vi "Curriculum Launcher.vi"(5 "Array of VISA Resources":refnum<visa-resource-name>[](array[refnum]), 7 "Device type":string[](array[string]), 8 "error in (no error)":errorcluster, 10 "Is the required hardware detected?":bool[](array[boolean]), 11 "Example File Paths":path[](array[path])) -> (0 "error out":errorcluster)   [LabVIEW 2020]
uses:
  <vilib>/Utility/sysdir.llb/System Directory Type.ctl
panel:
  in  "View Solution":bool
  in  "Multicolumn Listbox":i32(listbox)
  in  "Open Excercise Manual":bool
  in  "Open Button":bool
  # "If hardware is detected, the device references will be \npassed to the example."
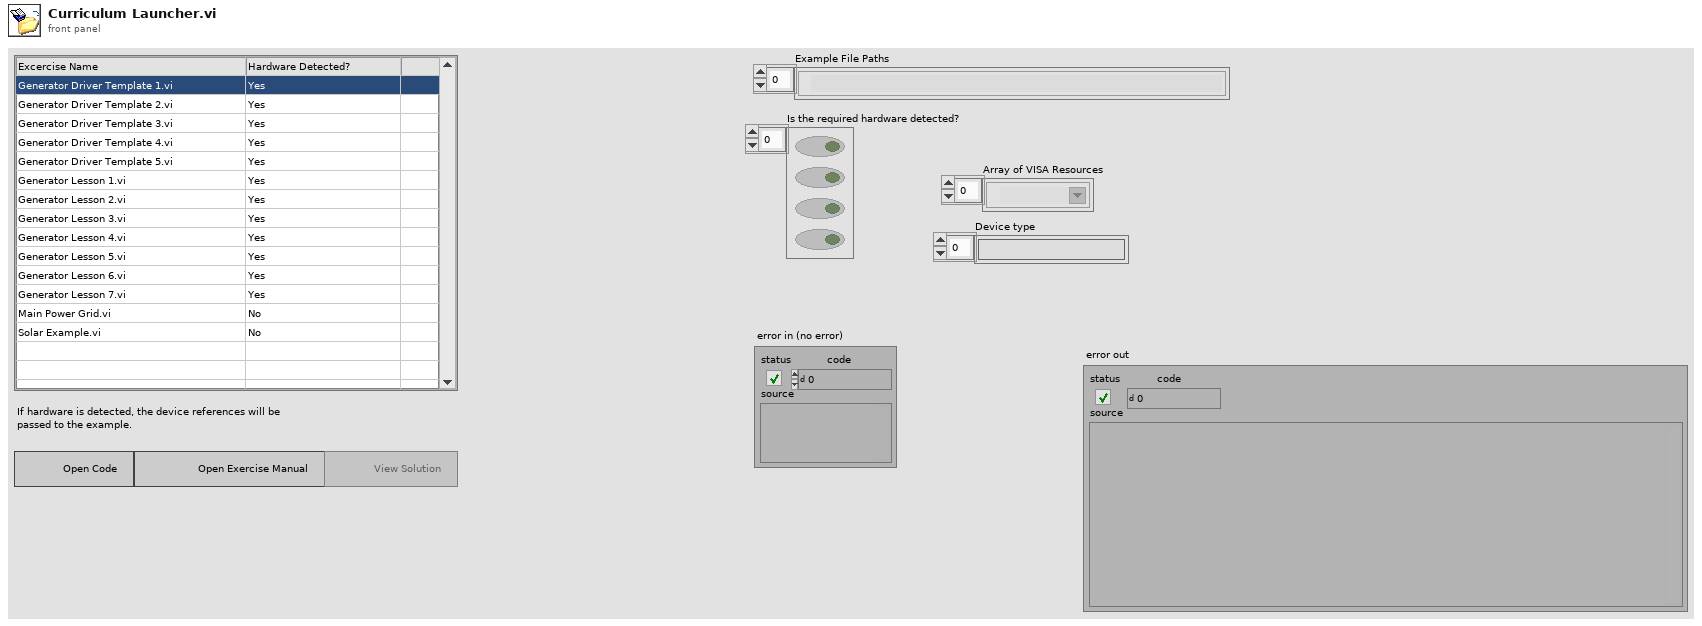
[diagram p1: front panel]
types:
  T1 = enum8{"Enabled", "Disabled", "Disabled and Grayed Out"}
  T2 = cluster{"Open Button":refnum<vi>, "Open Excercise Manual":refnum<vi>}
  T3 = enum32{"Invalid", "Standard", "Closed", "Hidden", "Minimized", "Maximized"}
  T4 = typedef "System Directory Type.ctl" = i32
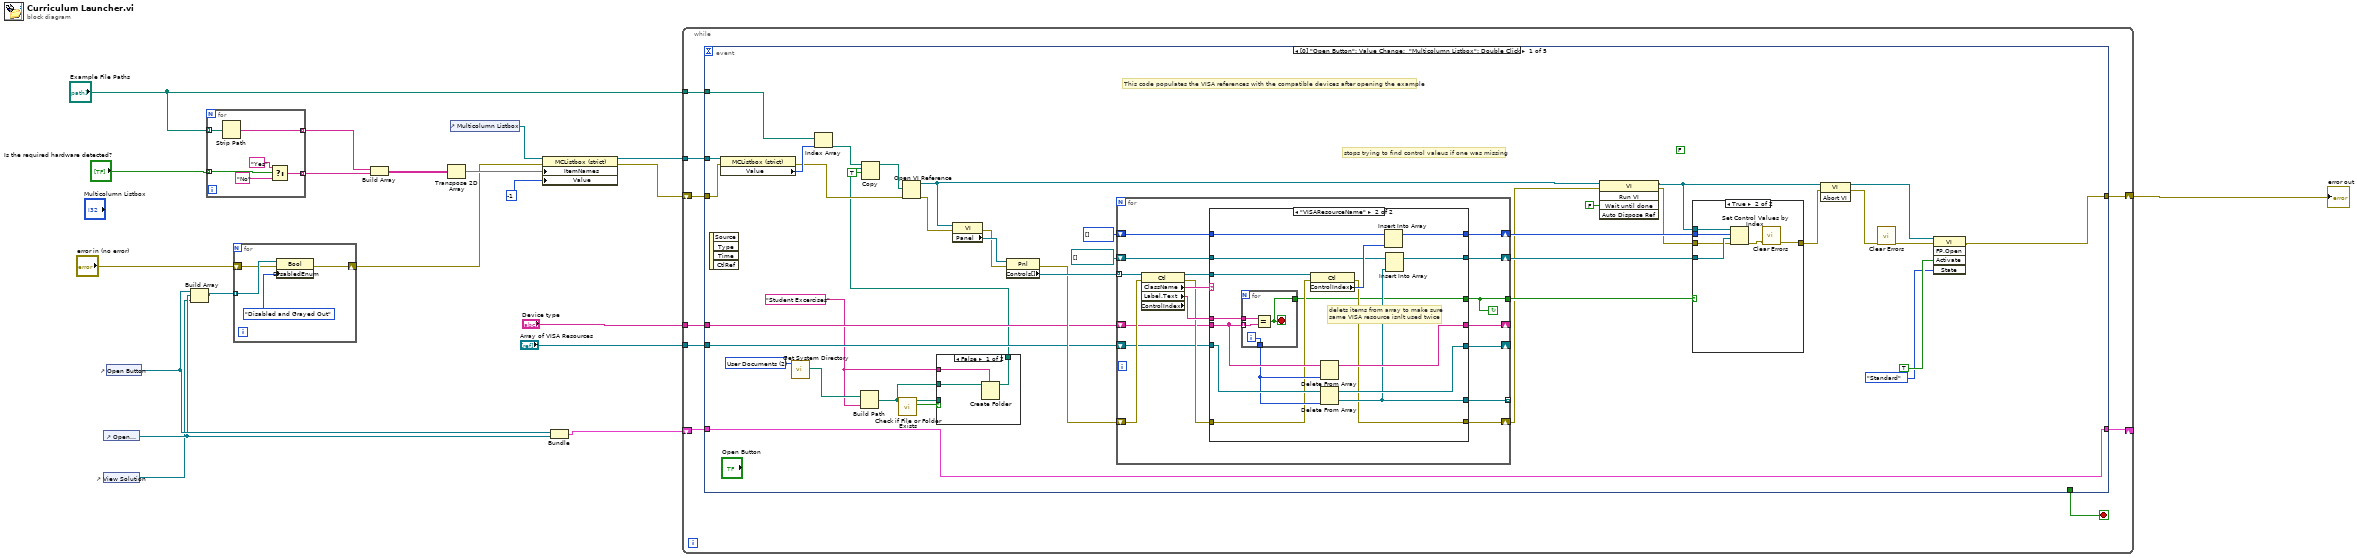
[diagram p0: block diagram]
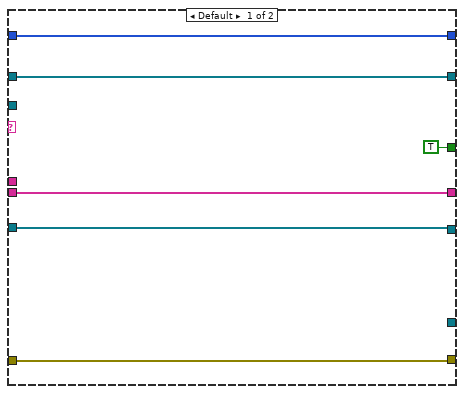
[diagram p4: hidden frame]
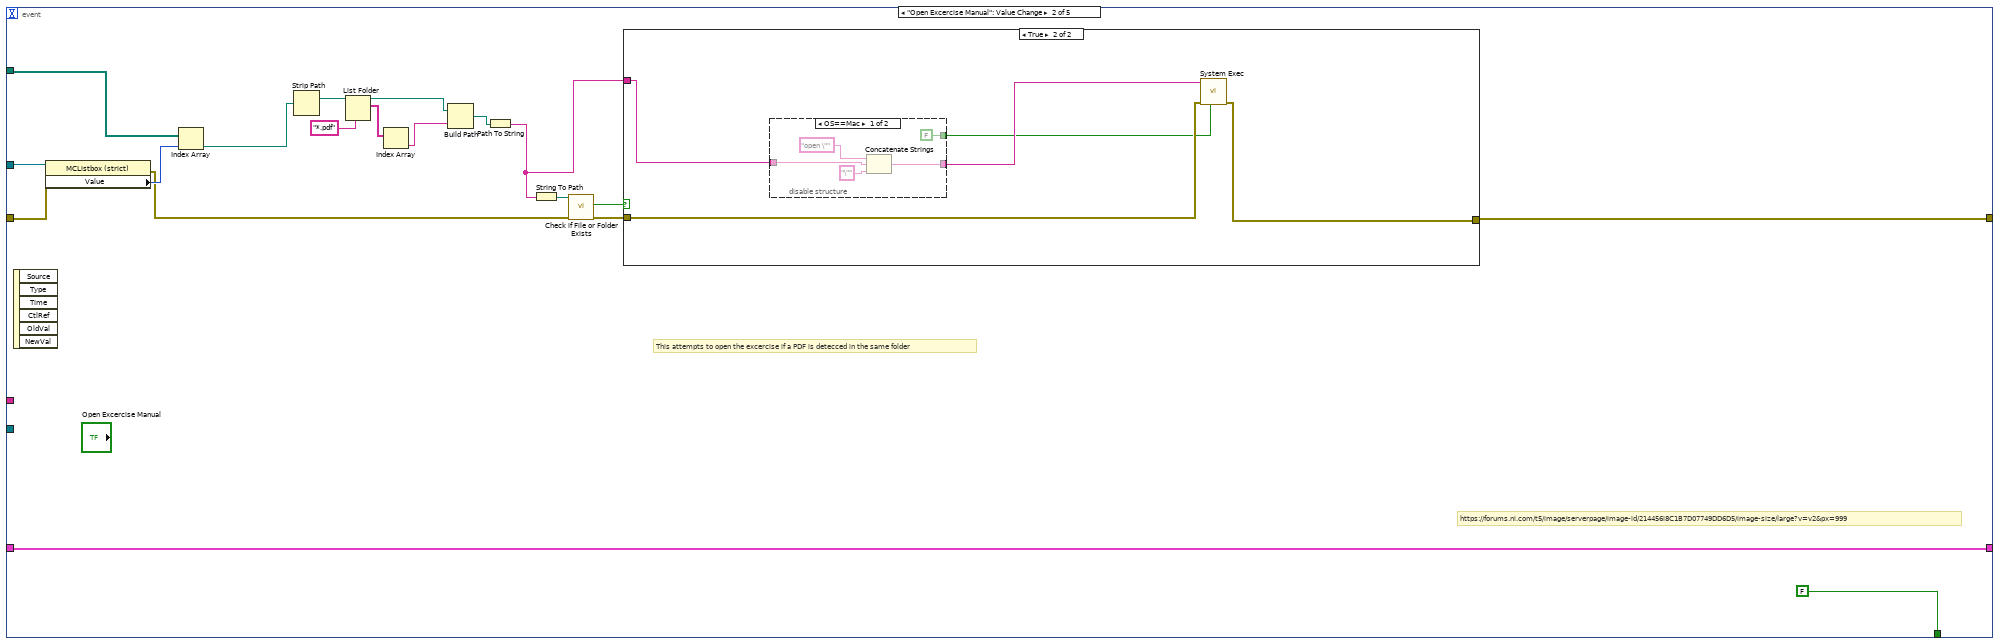
[diagram p5: hidden frame]
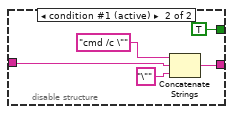
[diagram p7: hidden frame]
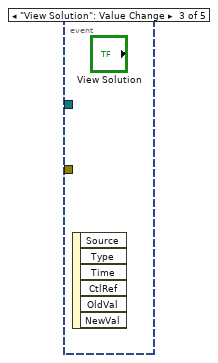
[diagram p8: hidden frame]
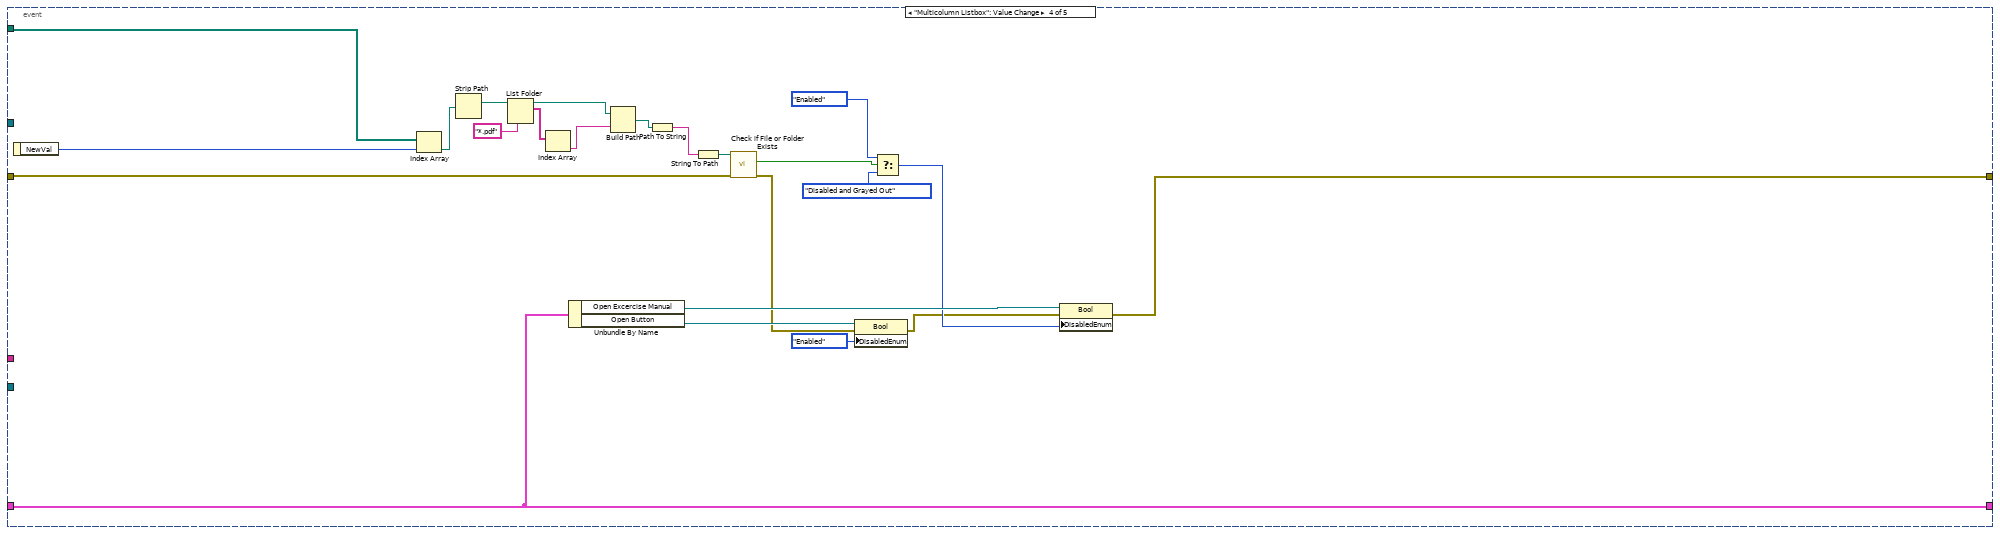
[diagram p9: hidden frame]
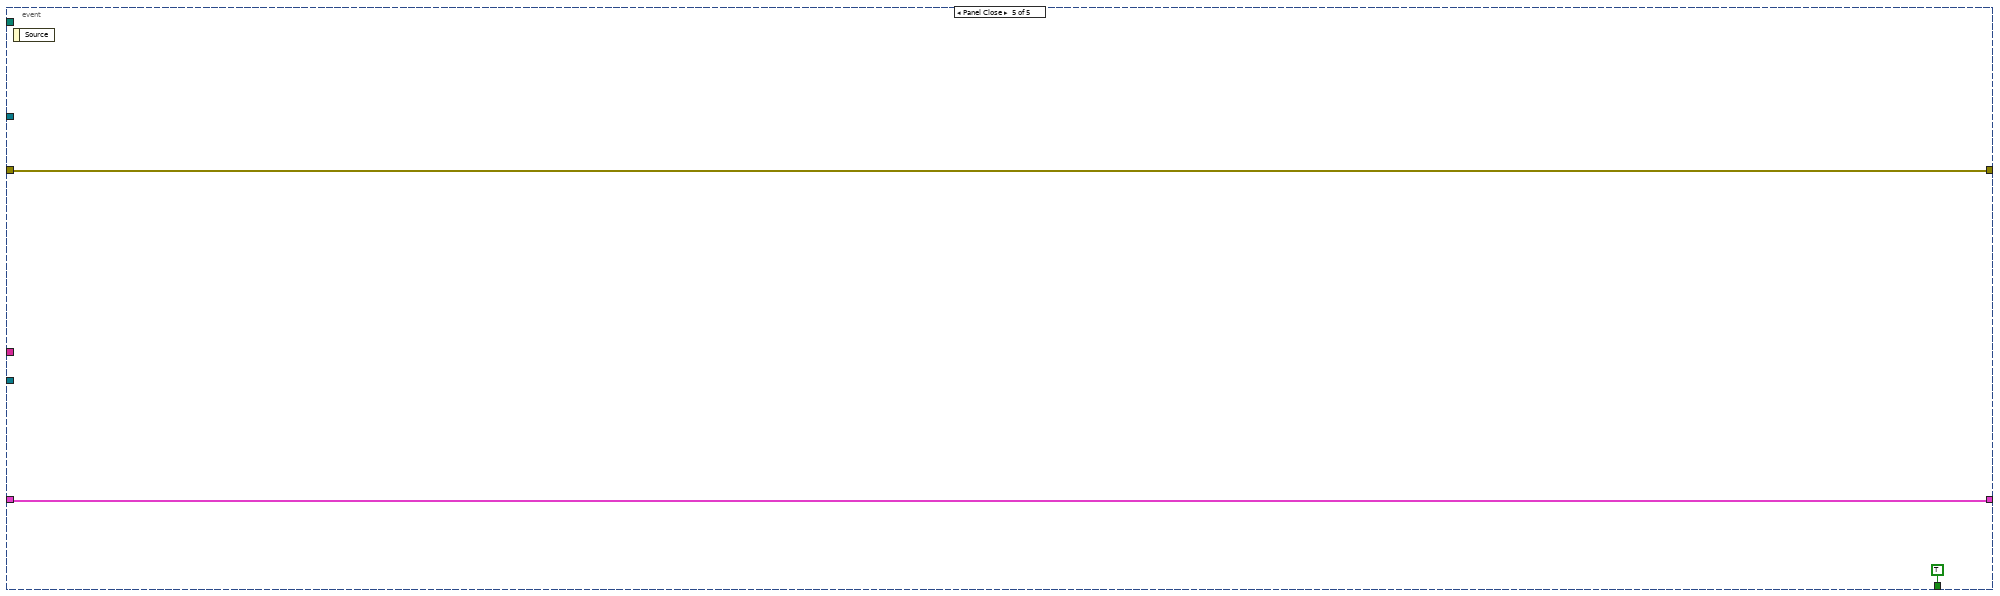
[diagram p10: hidden frame]
diagram:
  n1 = control-ref of="Open Excercise Manual"() -> (w13:refnum<vi>)
  n2 = control-ref of="View Solution"() -> (w1:refnum<vi>)
  n3 = control-ref of="Open Button"() -> (w14:refnum<vi>)
  n4 = Build Array(w14, w13, w1) -> (w12:refnum<vi>[])
  n5 = for {
    tunnel: "Example File Paths" -> [w26] mode=indexing
    tunnel: [w21] -> w9 mode=indexing
    tunnel: "Is the required hardware detected?" -> [w25] mode=indexing
    tunnel: [w22] -> w8 mode=indexing
    n6 = Strip Path(path=w26) -> (name=w21:string)  [unwired: 1 out]
    n7 = Select(t="Yes" ("concatenated string"), s=w25, f="No" ("concatenated string")) -> (s? t:f=w22:string)
  }
  n8 = for {
    tunnel: w12 -> [w29] mode=indexing
    shift-right: [w27] -> w2
    shift-left: "error in (no error)" -> [w28]
    n9 = property class="Bool"(reference=w29, error in=w28, "DisabledEnum"=T1."Disabled and Grayed Out" ("Disabled")) -> (error out=w27:errorcluster)  [unwired: 1 out]
  }
  n10 = Build Array(w9, w8) -> (w6:string[][])
  n11 = Transpose 2D Array(2D array=w6) -> (transposed array=w5:string[][])
  n12 = control-ref of="Multicolumn Listbox"() -> (w10:refnum<vi>)
  n13 = property on="Property Node" class="MCListbox (strict)"(reference=w10, error in=w2, "ItemNames"=w5, "Value"=-1) -> (reference out=w4:refnum<vi>, error out=w3:errorcluster)
  n14 = Bundle("Open Button"=w14, "Open Excercise Manual"=w13) -> (w15:T2)  [unwired: 1 in]
  n15 = while {
    tunnel: w4 -> [w38]
    tunnel: "Example File Paths" -> [w37]
    shift-right: [w36] -> w16
    shift-left: w3 -> [w39]
    tunnel: "Array of VISA Resources" -> [w35]
    tunnel: "Device type" -> [w34]
    shift-right: [w31] -> _
    shift-left: w15 -> [w32]
    stop <- w33 stop-if-true
    n16 = event shown="[0] \"Open Button\": Value Change;  \"Multicolumn Listbox\": Double Click" {
      selector: _ -> [_ _ _ _ _]
      dyn-events: _ -> [_ _ _ _ _]
      timeout: _ -> [_ _ _ _ _]
      tunnel: w39 -> [w76 w147 _ w177 w194]
      tunnel: w38 -> [w79 w149 _ _ _]
      tunnel: w37 -> [w77 w148 _ w179 _]
      tunnel: [w53 w152 _ w169 w194] -> w36
      tunnel: w35 -> [w69 _ _ _ _]
      tunnel: w34 -> [w68 _ _ _ _]
      tunnel: [_ FALSE _ _ TRUE] -> w33
      tunnel: w32 -> [w62 w134 _ w189 w192]
      tunnel: [w62 w134 _ w189 w192] -> w31
      event "Open Button": Value Change; "Multicolumn Listbox": Double Click {
        w41 = "Student Excercises" ("prompt (Create Folder)")
        w47 = T4 2 items=["User Home"=0, "User Desktop"=1, "User Documents"=2, "User Application Data"=3, "User Preferences"=4, "User Temporary"=5, "Public Documents"=6, "Public Application Data"=7, "Public Preferences"=8, "Public Cache"=13, "System Core Libraries"=9, "System Installed Libraries"=10, "Application Files"=11, "Boot Volume Root"=12] ("system directory type")
        (unwired) FALSE ("Wait Until Done")
        # "This code populates the VISA references with the compatible devices after opening the example"
        # "stops trying to find control valeus if one was missing"
        n17 = event-data() -> ()  [unwired: 1 in, 4 out]
        n18 = property on="Property Node" class="MCListbox (strict)"(reference=w79, error in=w76) -> (error out=w75:errorcluster, "Value"=w78:i32)  [unwired: 1 out]
        n19 = call <vilib>:"Get System Directory.vi"("system directory type"=w47) -> ("system directory"=w46:path)  [unwired: 10 in]
        n20 = Index Array(array=w77, index=w78) -> (element=w49:path)
        n21 = Build Path(base path=w46, name or relative path=w41) -> (appended path=w42:path)
        n22 = call <vilib>:"Check if File or Folder Exists.vi"("path"=w42) -> ("file or folder exists?"=w45:bool, "dup path"=w44:path)  [unwired: 8 in, 1 out]
        n23 = case shown="False" w45 {
          tunnel: w44 -> [_ w83]
          tunnel: [w81 w83] -> w43
          tunnel: w42 -> [w82 _]
          tunnel: w41 -> [w80 _]
          frame False {
            n24 = Create Folder(prompt (Create Folder)=w80, path (use dialog)=w82) -> (created path=w81:path)  [unwired: 1 in, 2 out]
          }
          frame True {
          }
        }
        n25 = Copy(9:TRUE ("overwrite (F)"), 10:w43, 11:w49) -> (3:w48:path)  [unwired: 2 in, 2 out]
        n26 = Open VI Reference(vi path=w48, error in (no error)=w75) -> (vi reference=w60:refnum<vi>, error out=w70:errorcluster)  [unwired: 4 in]
        n27 = property class="VI"(reference=w60, error in=w70) -> (error out=w72:errorcluster, "Panel"=w74:refnum<vi>)  [unwired: 1 out]
        n28 = property class="Pnl"(reference=w74, error in=w72) -> (error out=w71:errorcluster, "Controls[]"=w73:refnum<vi>[])  [unwired: 1 out]
        n29 = for {
          tunnel: w73 -> [w107] mode=indexing
          shift-right: [w102] -> w51
          shift-left: w71 -> [w105]
          shift-right: [w99] -> _
          shift-left: w68 -> [w100]
          shift-right: [w98] -> _
          shift-left: w69 -> [w101]
          tunnel: [w97] -> _ mode=indexing
          shift-right: [w95] -> w64
          shift-left: refnum<visa-resource-name>[] [] -> [w92]
          shift-right: [w94] -> w65
          shift-left: i32[] [] -> [w93]
          tunnel: [w91] -> w63
          stop <- w91 continue-if-true
          n30 = property class="Ctl" props=["ClassName", "Label", "Text", "ControlIndex"](reference=w107, error in=w105) -> (reference out=w96:refnum<vi>, error out=w103:errorcluster, "ClassName"=w106:string, "Label.Text"=w104:string)  [unwired: 1 out]
          n31 = case shown="\"VISAResourceName\"" w106 {
            tunnel: w104 -> [_ w129]
            tunnel: w103 -> [w111 w122]
            tunnel: [w111 w115] -> w102
            tunnel: w101 -> [w112 w128]
            tunnel: w100 -> [w113 w127]
            tunnel: [w113 w125] -> w99
            tunnel: [w112 w124] -> w98
            tunnel: [_ w120] -> w97
            tunnel: w96 -> [_ w123]
            tunnel: [w109 w119] -> w95
            tunnel: [w110 w118] -> w94
            tunnel: w93 -> [w110 w117]
            tunnel: w92 -> [w109 w116]
            tunnel: [TRUE w114] -> w91
            frame Default {
            }
            frame "VISAResourceName" {
              # "delets items from array to make sure\nsame VISA resource isnlt used twice"
              n32 = for {
                tunnel: w129 -> [w133]
                tunnel: w127 -> [w132] mode=indexing
                tunnel: [w131] -> w126
                tunnel: [w130] -> w114
                i -> [w131]
                stop <- w130 stop-if-true
                n33 = Equal?(x=w133, y=w132) -> (x = y?=w130:bool)
              }
              n34 = property class="Ctl"(reference=w123, error in=w122) -> (error out=w115:errorcluster, "ControlIndex"=w121:i32)  [unwired: 1 out]
              n35 = Delete From Array(array=w128, index=w126) -> (deleted portion=w120:refnum<visa-resource-name>, array with subset deleted=w124:refnum<visa-resource-name>[])  [unwired: 1 in]
              n36 = Delete From Array(array=w127, index=w126) -> (array with subset deleted=w125:string[])  [unwired: 1 in, 1 out]
              n37 = Insert Into Array(array=w117, new element=w121) -> (w118:i32[])  [unwired: 1 in]
              n38 = Insert Into Array(array=w116, new element=w120) -> (w119:refnum<visa-resource-name>[])  [unwired: 1 in]
            }
          }
        }
        n39 = invoke class="VI" method="Run VI"(reference=w60, error in=w51, "Wait until done"=FALSE ("Wait Until Done")) -> (reference out=w58:refnum<vi>, error out=w52:errorcluster)  [unwired: 2 in, 3 out]
        n40 = case shown="True" w63 {
          tunnel: w65 -> [_ w90]
          tunnel: w64 -> [_ w89]
          tunnel: [w84 w85] -> w59
          tunnel: w58 -> [_ w88]
          tunnel: w52 -> [w84 w87]
          frame False {
          }
          frame True {
            n41 = Set Control Values by Index(0:w88, 1:w90, 2:w89, 3:w87) -> (11:w86:errorcluster)
            n42 = call <vilib>:"Clear Errors.vi"("error in (no error)"=w86) -> ("error out"=w85:errorcluster)  [unwired: 5 in, 1 out]
          }
        }
        n43 = invoke class="VI" method="Abort VI"(reference=w58, error in=w59) -> (reference out=w57:refnum<vi>, error out=w54:errorcluster)  [unwired: 1 in, 1 out]
        n44 = call <vilib>:"Clear Errors.vi"("error in (no error)"=w54) -> ("error out"=w50:errorcluster)  [unwired: 5 in, 1 out]
        n45 = invoke class="VI" method="FP.Open"(reference=w57, error in=w50, "Activate"=TRUE ("Activate?"), "State"=T3."Standard") -> (error out=w53:errorcluster)  [unwired: 1 in, 4 out]
      }
      event "Open Excercise Manual": Value Change {
        # "https://forums.ni.com/t5/image/serverpage/image-id/214456i8C1B7D07749DD6D5/image-size/large?v=v2&px=999"
        # "This attempts to open the excercise if a PDF is detecced in the same folder"
        n46 = event-data() -> ()  [unwired: 1 in, 6 out]
        n47 = property on="Property Node" class="MCListbox (strict)"(reference=w149, error in=w147) -> (error out=w144:errorcluster, "Value"=w150:i32)  [unwired: 1 out]
        n48 = Index Array(array=w148, index=w150) -> (element=w142:path)
        n49 = Strip Path(path=w142) -> (stripped path=w141:path)  [unwired: 1 out]
        n50 = List Folder(path=w141, pattern="*.pdf") -> (path out=w138:path, filenames=w139:string[])  [unwired: 2 in, 2 out]
        n51 = Index Array(array=w139) -> (element=w137:string)  [unwired: 1 in]
        n52 = Build Path(base path=w138, name or relative path=w137) -> (appended path=w136:path)
        n53 = Path To String(path=w136) -> (string=w135:string)
        n54 = String To Path(string=w135) -> (path=w146:path)
        n55 = call <vilib>:"Check if File or Folder Exists.vi"("error in (no error)"=w144, "path"=w146) -> ("error out"=w143:errorcluster, "file or folder exists?"=w145:bool)  [unwired: 7 in, 1 out]
        n56 = case shown="True" w145 {
          tunnel: [w153 w158] -> w152
          tunnel: w135 -> [_ w156]
          tunnel: w143 -> [w153 w157]
          frame False {
          }
          frame True {
            n57 = disable-structure shown="OS==Mac" {
              disable-tunnel: w156 -> [w161 w166]
              disable-tunnel: [w160 w165] -> w155
              disable-tunnel: [FALSE ("run minimized? (F)") TRUE ("run minimized? (F)")] -> w154
              frame condition #0 {
                n58 = Concatenate Strings("open \"" ("string"), w161, "\"" ("string")) -> (w160:string)
              }
              frame condition #1 (active) {
                n59 = Concatenate Strings("cmd /c \"" ("string"), w166, "\"" ("string")) -> (w165:string)
              }
            }
            n60 = call <vilib>:"System Exec.vi"("run minimized? (F)"=w154, "error in (no error)"=w157, "command line"=w155) -> ("error out"=w158:errorcluster)  [unwired: 5 in, 3 out]
          }
        }
      }
      event "View Solution": Value Change {
        n61 = event-data() -> ()  [unwired: 1 in, 6 out]
      }
      event "Multicolumn Listbox": Value Change {
        n62 = event-data() -> ("NewVal"=w178:i32)  [unwired: 1 in]
        n63 = Index Array(array=w179, index=w178) -> (element=w187:path)
        n64 = Strip Path(path=w187) -> (stripped path=w186:path)  [unwired: 1 out]
        n65 = List Folder(path=w186, pattern="*.pdf") -> (path out=w183:path, filenames=w184:string[])  [unwired: 2 in, 2 out]
        n66 = Index Array(array=w184) -> (element=w182:string)  [unwired: 1 in]
        n67 = Unbundle By Name(w189) -> ("Open Excercise Manual"=w176:refnum<vi>, "Open Button"=w191:refnum<vi>)
        n68 = Build Path(base path=w183, name or relative path=w182) -> (appended path=w181:path)
        n69 = Path To String(path=w181) -> (string=w180:string)
        n70 = String To Path(string=w180) -> (path=w188:path)
        n71 = call <vilib>:"Check if File or Folder Exists.vi"("error in (no error)"=w177, "path"=w188) -> ("error out"=w171:errorcluster, "file or folder exists?"=w175:bool)  [unwired: 7 in, 1 out]
        n72 = property class="Bool"(reference=w191, error in=w171, "DisabledEnum"=T1."Enabled" ("Disabled")) -> (error out=w170:errorcluster)  [unwired: 1 out]
        n73 = Select(t=T1."Enabled" ("Disabled"), s=w175, f=T1."Disabled and Grayed Out" ("Disabled")) -> (s? t:f=w172:T1)
        n74 = property class="Bool"(reference=w176, error in=w170, "DisabledEnum"=w172) -> (error out=w169:errorcluster)  [unwired: 1 out]
      }
      event Panel Close {
        n75 = event-data() -> ()  [unwired: 1 in, 1 out]
      }
    }
  }
  "error out" <- w16
